vi "VIH - CHM Project - Write HHP File.vi"(7 "Abs CHM Path (F)":bool, 8 "error in":errorcluster, 9 "Files":T1, 10 "Target HHP File":path, 11 "Template HHP File":path) -> (0 "error out":errorcluster)   [LabVIEW 2014]
doc: "::: VI Helpeks :::\nCopyright (c) 2000-2026 Konstantin Shifershteyn. All rights reserved."
panel:
  # "VI Helpeks\nCopyright (c) 2012-2026 Konstantin Shifershteyn"
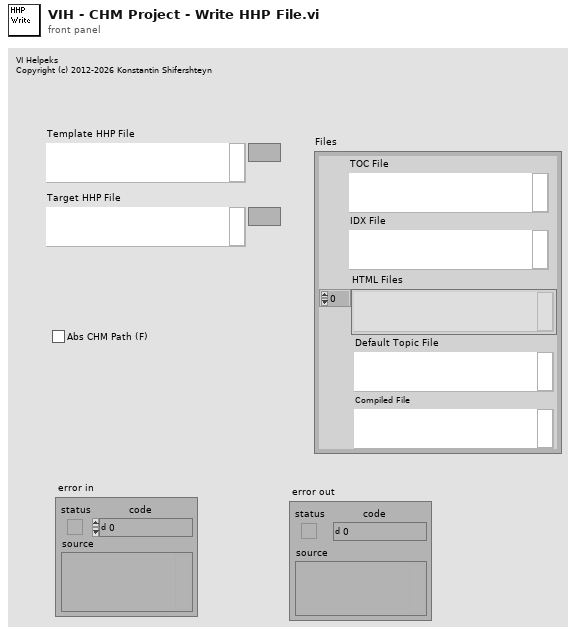
[diagram p1: front panel]
types:
  T1 = cluster{"TOC File":path, "IDX File":path, "HTML Files":path[], "Default Topic File":path, "Compiled File":path}
  T2 = typedef "VIH - CHM Project - HHP Support - Queue Refnum.ctl" = refnum<queue>
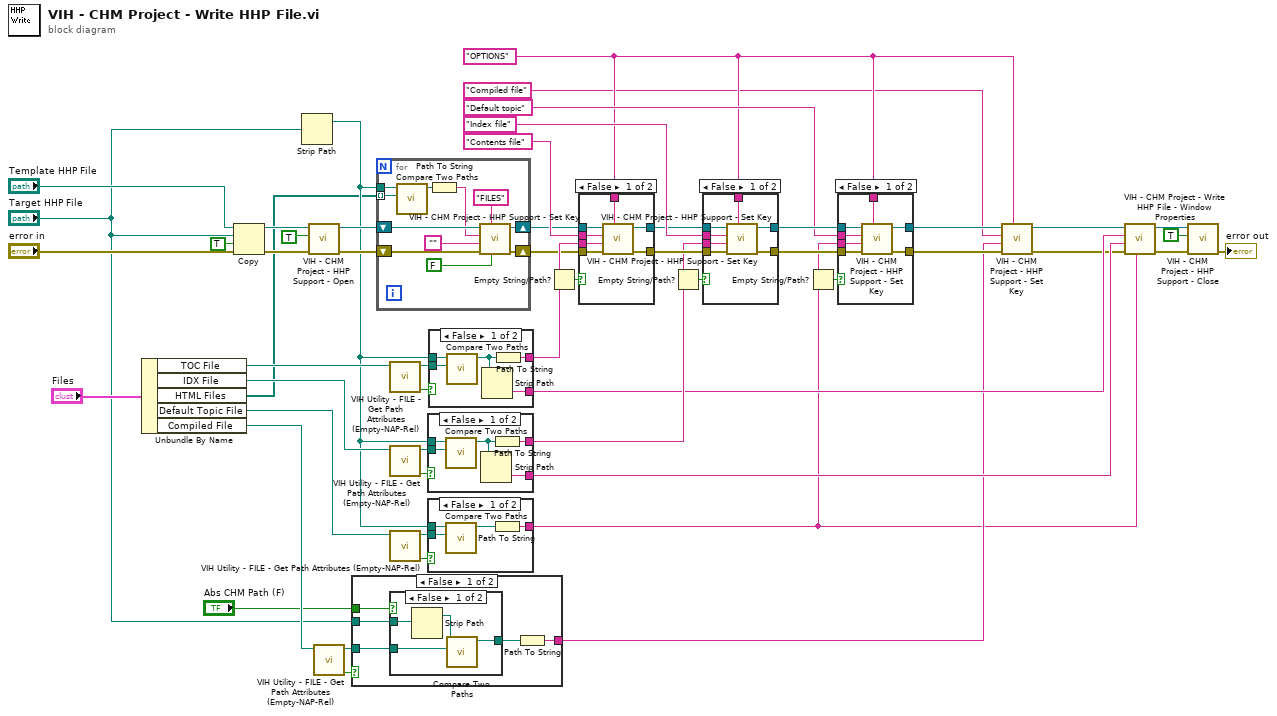
[diagram p0: block diagram]
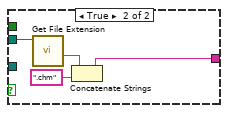
[diagram p3: hidden frame]
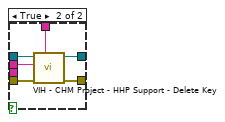
[diagram p5: hidden frame]
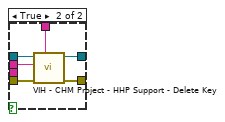
[diagram p7: hidden frame]
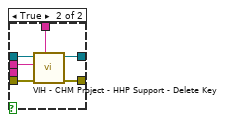
[diagram p9: hidden frame]
diagram:
  w15 = "OPTIONS" ("Section")
  n1 = Unbundle By Name("Files") -> ("TOC File"=w26:path, "IDX File"=w25:path, "HTML Files"=w3:path[], "Default Topic File"=w18:path, "Compiled File"=w9:path)
  n2 = Copy(8:"error in", 9:TRUE, 10:"Target HHP File", 11:"Template HHP File") -> (0:w50:errorcluster, 3:w52:path)  [unwired: 1 in, 1 out]
  n3 = Strip Path(path="Target HHP File") -> (stripped path=w8:path)  [unwired: 1 out]
  n4 = call "VIH - CHM Project - HHP Support - Open.vi"("error in"=w50, "must exist (F)"=TRUE, "Config File"=w52) -> ("error out"=w46:errorcluster, "queue out"=w47:T2)  [unwired: 7 in]
  n5 = call "VIH Utility - FILE - Get Path Attributes (Empty-NAP-Rel).vi"("Path"=w9) -> ("Not A Path or Empty path"=w10:bool, "dup Path"=w11:path)  [unwired: 6 in, 3 out]
  n6 = case shown="False" w10 {
    tunnel: w11 -> [w58 _]
    tunnel: [w57 w64] -> w6
    tunnel: "Target HHP File" -> [w55 w65]
    tunnel: "Abs CHM Path (F)" -> [w54 _]
    frame False {
      n7 = case shown="False" w54 {
        tunnel: w58 -> [w62 w63]
        tunnel: [w61 w63] -> w56
        tunnel: w55 -> [w60 _]
        frame False {
          n8 = Strip Path(path=w60) -> (stripped path=w59:path)  [unwired: 1 out]
          n9 = call <vilib>:"Compare Two Paths.vi"("Path 2"=w62, "Path 1"=w59) -> ("Relative Path from 1 to 2"=w61:path)  [unwired: 6 in, 3 out]
        }
        frame True {
        }
      }
      n10 = Path To String(path=w56) -> (string=w57:string)
    }
    frame True {
      n11 = call <vilib>:"Get File Extension.vi"("file"=w65) -> ("filename without extension"=w66:string)  [unwired: 7 in, 3 out]
      n12 = Concatenate Strings(w66, ".chm" ("string")) -> (w64:string)
    }
  }
  n13 = for {
    shift-right: [w76] -> w5
    shift-left: w47 -> [w78]
    shift-right: [w74] -> w4
    shift-left: w46 -> [w77]
    tunnel: w8 -> [w71]
    tunnel: w3 -> [w70] mode=indexing
    n14 = call <vilib>:"Compare Two Paths.vi"("Path 2"=w70, "Path 1"=w71) -> ("Relative Path from 1 to 2"=w69:path)  [unwired: 6 in, 3 out]
    n15 = Path To String(path=w69) -> (string=w68:string)
    n16 = call "VIH - CHM Project - HHP Support - Set Key.vi"("key/value separator (T)"=FALSE, "Section"="FILES", "error in"=w77, "Value"="", "Key"=w68, "queue"=w78) -> ("error out"=w74:errorcluster, "dup queue"=w76:T2)  [unwired: 4 in]
  }
  n17 = call "VIH Utility - FILE - Get Path Attributes (Empty-NAP-Rel).vi"("Path"=w26) -> ("Not A Path or Empty path"=w28:bool, "dup Path"=w31:path)  [unwired: 6 in, 3 out]
  n18 = call "VIH Utility - FILE - Get Path Attributes (Empty-NAP-Rel).vi"("Path"=w25) -> ("Not A Path or Empty path"=w29:bool, "dup Path"=w30:path)  [unwired: 6 in, 3 out]
  n19 = call "VIH Utility - FILE - Get Path Attributes (Empty-NAP-Rel).vi"("Path"=w18) -> ("Not A Path or Empty path"=w20:bool, "dup Path"=w19:path)  [unwired: 6 in, 3 out]
  n20 = case shown="False" w29 {
    tunnel: w8 -> [w83 _]
    tunnel: w30 -> [w82 _]
    tunnel: [w81 _] -> w36
    tunnel: [w79 _] -> w32
    frame False {
      n21 = call <vilib>:"Compare Two Paths.vi"("Path 2"=w82, "Path 1"=w83) -> ("Relative Path from 1 to 2"=w80:path)  [unwired: 6 in, 3 out]
      n22 = Strip Path(path=w80) -> (name=w79:string)  [unwired: 1 out]
      n23 = Path To String(path=w80) -> (string=w81:string)
    }
    frame True {
    }
  }
  n24 = case shown="False" w20 {
    tunnel: w8 -> [w87 _]
    tunnel: w19 -> [w86 _]
    tunnel: [w85 _] -> w1
    frame False {
      n25 = call <vilib>:"Compare Two Paths.vi"("Path 2"=w86, "Path 1"=w87) -> ("Relative Path from 1 to 2"=w84:path)  [unwired: 6 in, 3 out]
      n26 = Path To String(path=w84) -> (string=w85:string)
    }
    frame True {
    }
  }
  n27 = case shown="False" w28 {
    tunnel: w8 -> [w92 _]
    tunnel: w31 -> [w91 _]
    tunnel: [w90 _] -> w41
    tunnel: [w88 _] -> w33
    frame False {
      n28 = call <vilib>:"Compare Two Paths.vi"("Path 2"=w91, "Path 1"=w92) -> ("Relative Path from 1 to 2"=w89:path)  [unwired: 6 in, 3 out]
      n29 = Strip Path(path=w89) -> (name=w88:string)  [unwired: 1 out]
      n30 = Path To String(path=w89) -> (string=w90:string)
    }
    frame True {
    }
  }
  n31 = Empty String/Path?(string/path=w41) -> (empty?=w42:bool)
  n32 = case shown="False" w42 {
    tunnel: w5 -> [w99 w105]
    tunnel: w15 -> [w98 w103]
    tunnel: w4 -> [w97 w102]
    tunnel: w41 -> [w96 _]
    tunnel: "Contents file" ("Key") -> [w95 w104]
    tunnel: [w94 w100] -> w38
    tunnel: [w93 w101] -> w37
    frame False {
      n33 = call "VIH - CHM Project - HHP Support - Set Key.vi"("Section"=w98, "error in"=w97, "Value"=w96, "Key"=w95, "queue"=w99) -> ("error out"=w93:errorcluster, "dup queue"=w94:T2)  [unwired: 5 in]
    }
    frame True {
      n34 = call "VIH - CHM Project - HHP Support - Delete Key.vi"("Section"=w103, "error in"=w102, "Key"=w104, "queue"=w105) -> ("error out"=w101:errorcluster, "dup queue"=w100:T2)  [unwired: 6 in]
    }
  }
  n35 = Empty String/Path?(string/path=w36) -> (empty?=w40:bool)
  n36 = case shown="False" w40 {
    tunnel: w38 -> [w112 w118]
    tunnel: w15 -> [w111 w116]
    tunnel: w37 -> [w110 w115]
    tunnel: w36 -> [w109 _]
    tunnel: "Index file" ("Key") -> [w108 w117]
    tunnel: [w107 w113] -> w23
    tunnel: [w106 w114] -> w22
    frame False {
      n37 = call "VIH - CHM Project - HHP Support - Set Key.vi"("Section"=w111, "error in"=w110, "Value"=w109, "Key"=w108, "queue"=w112) -> ("error out"=w106:errorcluster, "dup queue"=w107:T2)  [unwired: 5 in]
    }
    frame True {
      n38 = call "VIH - CHM Project - HHP Support - Delete Key.vi"("Section"=w116, "error in"=w115, "Key"=w117, "queue"=w118) -> ("error out"=w114:errorcluster, "dup queue"=w113:T2)  [unwired: 6 in]
    }
  }
  n39 = Empty String/Path?(string/path=w1) -> (empty?=w24:bool)
  n40 = case shown="False" w24 {
    tunnel: w23 -> [w125 w131]
    tunnel: w15 -> [w124 w129]
    tunnel: w22 -> [w123 w128]
    tunnel: w1 -> [w122 _]
    tunnel: "Default topic" ("Key") -> [w121 w130]
    tunnel: [w120 w126] -> w17
    tunnel: [w119 w127] -> w14
    frame False {
      n41 = call "VIH - CHM Project - HHP Support - Set Key.vi"("Section"=w124, "error in"=w123, "Value"=w122, "Key"=w121, "queue"=w125) -> ("error out"=w119:errorcluster, "dup queue"=w120:T2)  [unwired: 5 in]
    }
    frame True {
      n42 = call "VIH - CHM Project - HHP Support - Delete Key.vi"("Section"=w129, "error in"=w128, "Key"=w130, "queue"=w131) -> ("error out"=w127:errorcluster, "dup queue"=w126:T2)  [unwired: 6 in]
    }
  }
  n43 = call "VIH - CHM Project - HHP Support - Set Key.vi"("Section"=w15, "error in"=w14, "Value"=w6, "Key"="Compiled file", "queue"=w17) -> ("error out"=w13:errorcluster, "dup queue"=w16:T2)  [unwired: 5 in]
  n44 = call "VIH - CHM Project - Write HHP File - Window Properties.vi"("Default Topic"=w1, "error in"=w13, "Index Filename"=w32, "TOC Filename"=w33, "queue"=w16) -> ("error out"=w34:errorcluster, "dup queue"=w35:T2)  [unwired: 5 in]
  n45 = call "VIH - CHM Project - HHP Support - Close.vi"("error in"=w34, "write file (F)"=TRUE, "queue"=w35) -> ("error out"=→"error out":errorcluster)  [unwired: 8 in]
